vi "Transfer Images Data to UI.vi"(0 "fpga interface in":refnum<k20>, 1 "'stop' notifier":refnum<notifier>, 3 "measure call context in":refnum<class "Measure Call Context.lvclass">, 5 "Active Channel":string[](array[string]), 11 "error in":errorcluster, 12 "References":T1, 13 "raw display notifier":refnum<notifier>) -> (4 "fpga interface out":refnum<k20>, 15 "error out":errorcluster)   [LabVIEW 2025, in "Automotive Vision.lvclass"]
doc: "Handles frame grabbing, and prepare data for sendig it to the UI."
uses:
  Automotive Vision.lvclass
  Automotive Vision.lvclass/Automotive Vision.ctl
  <vilib>/rvi/interface/nirviReadWriteControl/nirviReadWriteControl.xnode
  deps/NI148X/Getting Started/Host/Common/GettingStarted_Common_148X_Host.lvlib
  deps/NI148X/Getting Started/Host/Common/Types/148x_Common_FPGA_Reference.ctl
  NiFpgaLv.dll
  <vilib>/Utility/error.llb/Error Cluster From Error Code.vi
  <vilib>/rvi/interface/Simulation/niFpgaSimulationCallBeginRW.vi
  <vilib>/rvi/errors/niLvFpgaAdjustHostInterfaceError.vi
  <vilib>/Plug-In SDKs/Measurements/Measure Call Context/Measure Call Context.lvclass
  <instrlib>/FlexRIO/CSI-2/v2/Common/Types/LLP Data Type.ctl
  <instrlib>/FlexRIO/CSI-2/v2/Common/NI CSI-2 API Common v2.lvlib
  Automotive-Vision OOB Data Transfer/Automotive-Vision OOB Data Transfer.lvlib
  Measurement Results.ctl
  <vilib>/vision/Image Controls.llb/IMAQ Image.ctl
  deps/NI148X/Getting Started/Host/Common/Types/RAW Interpretation for Display.ctl
  deps/NI148X/Getting Started/Host/Common/Types/Serial Channel Display Parameters.ctl
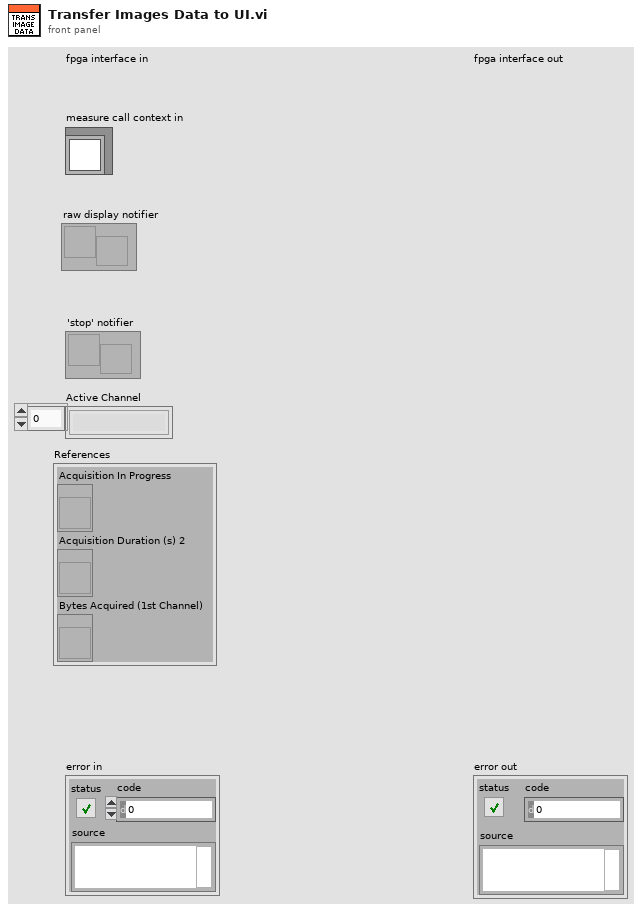
[diagram p1: front panel]
types:
  T1 = cluster{"Acquisition In Progress":refnum<vi>, "Acquisition Duration (s) 2":refnum<vi>, "Bytes Acquired (1st Channel)":refnum<vi>}
  T2 = typedef "NI CSI-2 API Common v2.lvlib/LLP Data Type.ctl" = enum8{"Frame Start", "Frame End", "Line Start", "Line End", "End of Transmission", "Reserved 0", "Reserved 1", "Reserved 2", "Generic Short Packet 1", "Generic Short Packet 2", "Generic Short Packet 3", "Generic Short Packet 4", "Generic Short Packet 5", "Generic Short Packet 6", "Generic Short Packet 7", "Generic Short Packet 8", "Null", "Blanking Data", "Embedded 8-bit non Image Data", "Generic Long Packet 1", "Generic Long Packet 2", "Generic Long Packet 3", "Generic Long Packet 4", "Reserved 3", "YUV420 8-bit", "YUV420 10-bit", "Legacy YUV420 8-bit", "Reserved 4", "YUV420 8-bit Chroma Shifted", "YUV420 10-bit Chroma Shifted", "YUV422 8-bit", "YUV422 10-bit", "RGB444", "RGB555", "RGB565", "RGB666", "RGB888", "Reserved 5", "Reserved 6", "RAW 24", "RAW 6", "RAW 7", "RAW 8", "RAW 10", "RAW 12", "RAW 14", "RAW 16", "RAW 20", "User Defined 8-bit Data 1", "User Defined 8-bit Data 2", "User Defined 8-bit Data 3", "User Defined 8-bit Data 4", "User Defined 8-bit Data 5", "User Defined 8-bit Data 6", "User Defined 8-bit Data 7", "User Defined 8-bit Data 8", "USL Command", "Reserved 7", "Reserved 8", "Reserved 9", "Reserved 10", "Reserved 11", "Reserved 12", "LRTE EPD Spacer"}
  T3 = cluster{"serial channel":fxp<+,3,3>, "frame number":u16, "data type":T2, "width":u16, "height":u16, "image bytes":u32, "total bytes":u32, "little endian":bool, "Status":string}
  T4 = typedef "GettingStarted_Common_148X_Host.lvlib/148x_Common_FPGA_Reference.ctl" = refnum<k20>
  T5 = typedef "GettingStarted_Common_148X_Host.lvlib/Serial Channel Display Parameters.ctl" = cluster{"images":cluster{"grayscale":T6, "color":T6}, "RAW parameters":cluster{"interpretation":T7, "bayer parameters":cluster{"pattern":i32, "algorithm":i32, "red gain":dbl, "green gain":dbl, "blue gain":dbl}}}
  T6 = typedef "IMAQ Image.ctl" = refnum<image>
  T7 = typedef "GettingStarted_Common_148X_Host.lvlib/RAW Interpretation for Display.ctl" = enum16{"Grayscale", "Bayer", "RGB", "YUV422", "YUV420", "Legacy YUV420"}
  T8 = typedef "GettingStarted_Common_148X_FPGA.lvlib/Image Metadata.ctl" = cluster{"serial channel":fxp<+,3,3>, "frame number":u16, "data type":T2, "width":u16, "height":u16, "image bytes":u32, "total bytes":u32, "little endian":bool}
  T9 = typedef "Automotive-Vision OOB Data Transfer.lvlib/OOB to Logic Data.ctl" = cluster{"PauseResume":bool, "ExportPath":string, "ExportType":u16, "Export":bool}
  T10 = typedef "Automotive Vision.lvclass/Measurement Results.ctl" = cluster{"ACQ. IN PROGRESS":bool, "IMAGE PIXEL DATA":u32[], "ACQ. DURATION (s)":dbl, "SOURCE RATE (fps)":dbl, "BYTES ACQUIRED":u64, "FRAME COUNT":u64, "POC VOLTAGE (V)":dbl, "POC CURRENT (A)":dbl, "ERROR":bool, "STATE MESSAGE":string, "IMAGE DATA":string, "OOB gRPC Port":i32, "HEIGHT":u64, "WIDTH":u64}
  T11 = cluster{"image pixel data fifo overflow":bool, "image metadata fifo overflow":bool}[]
  T12 = cluster{"image pixel data fifo overflow":bool, "image metadata fifo overflow":bool}
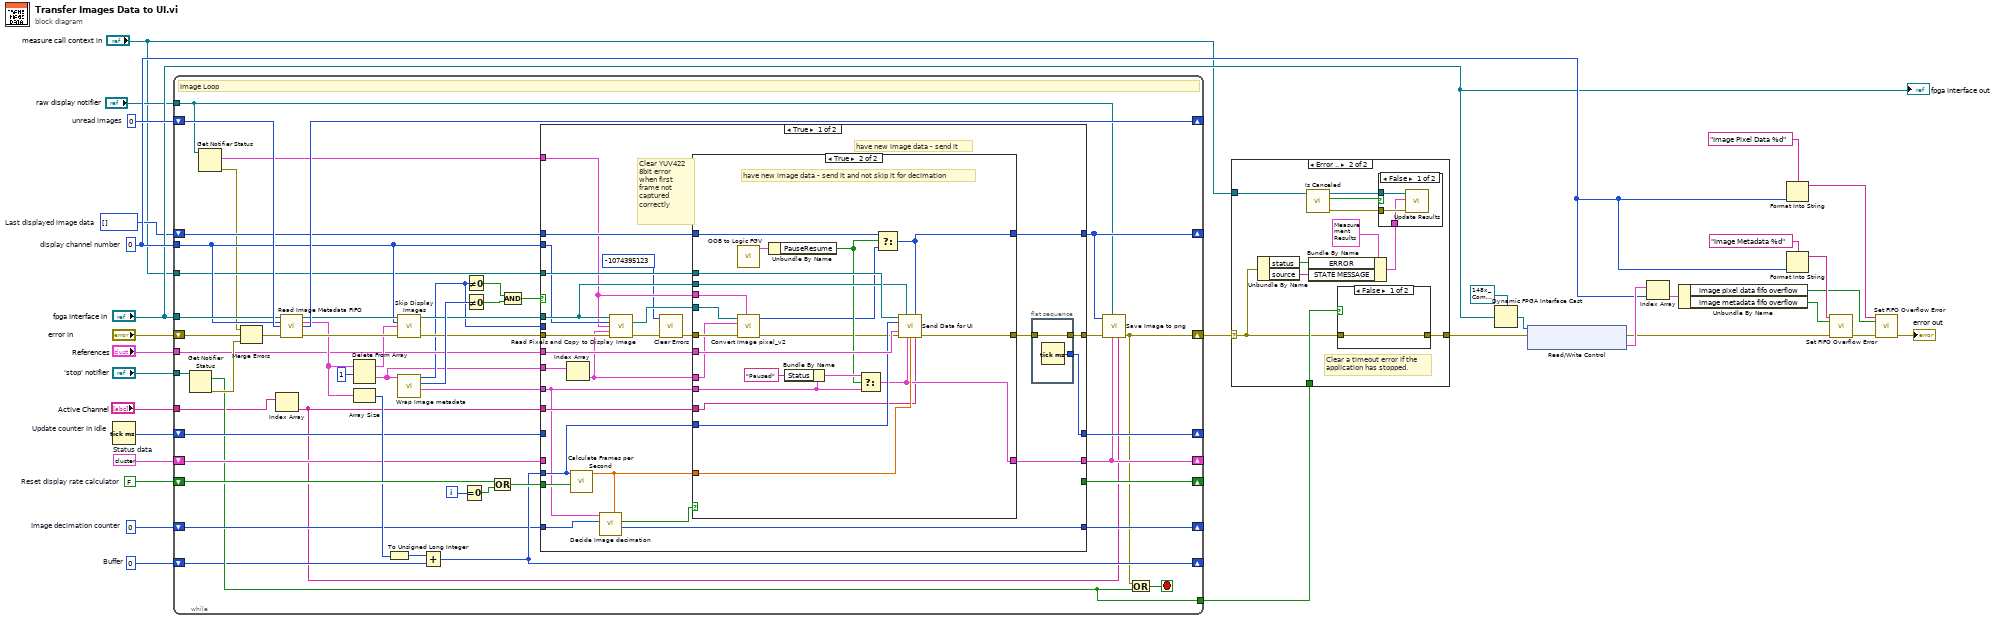
[diagram p0: block diagram]
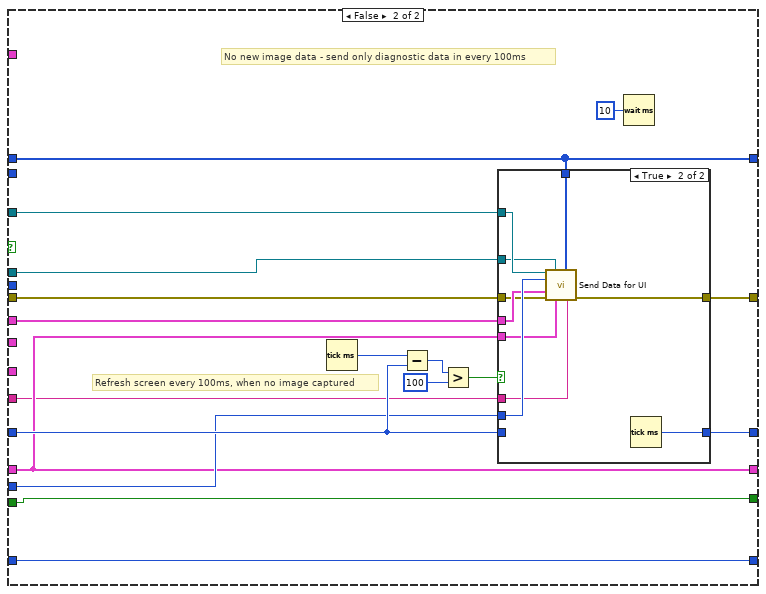
[diagram p3: hidden frame]
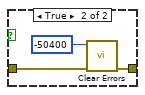
[diagram p7: hidden frame]
diagram:
  w4 = T3 {"serial channel"=0.0, "frame number"=0, "data type"=enum."Frame Start", "width"=0, "height"=0, "image bytes"=0, "total bytes"=0, "little endian"=FALSE, "Status"="Ready for Acquisition"}  # Status data
  w22 = 0  # display channel number
  w7 = u32 0  # Image decimation counter
  w8 = u32[] []  # Last displayed image data
  w14 = u32 0  # Buffer
  w15 = FALSE  # Reset display rate calculator
  w31 = u32 0  # unread images
  n1 = Tick Count (ms) "Update counter in Idle"() -> (millisecond timer value=w9:u32)
  n2 = while {
    shift-right: [w38] -> w13
    shift-left: "error in" -> [w56]
    tunnel: "fpga interface in" -> [w59]
    shift-right: [w79] -> _
    shift-left: w31 -> [w70]
    tunnel: w22 -> [w55]
    shift-right: [w74] -> _
    shift-left: w15 -> [w71]
    shift-right: [w61] -> _
    shift-left: w14 -> [w42]
    tunnel: [w44] -> w11
    tunnel: "'stop' notifier" -> [w58]
    shift-right: [w53] -> _
    shift-left: w9 -> [w54]
    shift-right: [w41] -> _
    shift-left: w8 -> [w52]
    shift-right: [w50] -> _
    shift-left: w7 -> [w51]
    tunnel: "References" -> [w49]
    tunnel: "measure call context in" -> [w48]
    shift-right: [w39] -> _
    shift-left: w4 -> [w47]
    tunnel: "raw display notifier" -> [w35]
    tunnel: "Active Channel" -> [w37]
    i -> [w78]
    stop <- w80 stop-if-true
    # "Image Loop"
    n3 = Get Notifier Status(notifier=w58) -> (current notification=w44:bool, error out=w81:errorcluster)  [unwired: 1 in, 3 out]
    n4 = Get Notifier Status(notifier=w35) -> (current notification=w33:T5[], error out=w34:errorcluster)  [unwired: 1 in, 3 out]
    n5 = Merge Errors(w34, w56, w81) -> (w57:errorcluster)
    n6 = Index Array(array=w37) -> (element=w36:string)  [unwired: 1 in]
    n7 = call "Read Image Metadata FIFO.vi"("fpga inteface in"=w59, "display channel number"=w55, "number of images"=w70, "error in (no error)"=w57) -> ("fpga interface out"=w67:refnum<k20>, "image metadata"=w60:T8[], "images remaining"=w79:u32, "error out"=w64:errorcluster)  [unwired: 8 in]
    n8 = Delete From Array(array=w60, length=1) -> (deleted portion=w32:T8[], array with subset deleted=w63:T8[])  [unwired: 1 in]
    n9 = Array Size(array=w60) -> (size(s)=w62:i32)
    n10 = To Unsigned Long Integer(number=w62) -> (unsigned 32bit integer=w43:u32)
    n11 = call "Skip Display Images.vi"("fpga interface in"=w67, "display channel number"=w55, "image metadata"=w63, "error in (no error)"=w64) -> ("fpga interface out"=w66:refnum<k20>, "error out"=w65:errorcluster)  [unwired: 10 in]
    n12 = call "Wrap Image metadata.vi"("image metadata"=w32) -> ("element"=w46:T3, "Numeric"=w69:i32, "total bytes"=w45:u32)  [unwired: 8 in]
    n13 = Add(x=w43, y=w42) -> (x+y=w61:u32)
    n14 = Equal To 0?(x=w78) -> (x = 0?=w72:bool)
    n15 = Not Equal To 0?(x=w45) -> (x != 0?=w76:bool)
    n16 = Not Equal To 0?(x=w69) -> (x != 0?=w77:bool)
    n17 = Compound Arithmetic op=OR(w71, w72) -> (w73:bool)
    n18 = Compound Arithmetic op=AND(w76, w77) -> (w75:bool)
    n19 = case shown="True" w75 {
      tunnel: w65 -> [w93 w136]
      tunnel: w66 -> [w92 w134]
      tunnel: w55 -> [w91 _]
      tunnel: [w105 w143] -> w40
      tunnel: w73 -> [w96 w150]
      tunnel: [_ w150] -> w74
      tunnel: w61 -> [w102 w140]
      tunnel: w45 -> [_ _]
      tunnel: w46 -> [w86 _]
      tunnel: w48 -> [w107 w137]
      tunnel: w49 -> [w106 w151]
      tunnel: w54 -> [_ w142]
      tunnel: [w104 w144] -> w53
      tunnel: w52 -> [w101 w141]
      tunnel: [w103 w141] -> w41
      tunnel: w51 -> [w100 w139]
      tunnel: [w99 w139] -> w50
      tunnel: w47 -> [_ w138]
      tunnel: [w97 w138] -> w39
      tunnel: w36 -> [w95 w135]
      tunnel: w33 -> [w87 _]
      tunnel: w32 -> [w90 _]
      frame True {
        # "Clear YUV422 8bit error when first frame not captured correctly"
        # "have new image data - send it"
        n20 = Index Array(array=w90) -> (element=w89:T8)  [unwired: 1 in]
        n21 = call <vilib>:"Calculate Frames per Second.vi"("Reset"=w96, "Buffer Number"=w102) -> ("Acquired Frames/s"=w85:dbl)  [unwired: 7 in, 2 out]
        n22 = call "Decide Image decimation.vi"("FPS"=w85, "Image decimation counter in"=w100, "element in"=w86) -> ("Image decimation counter out"=w99:u32, "send current image data"=w98:bool)  [unwired: 7 in]
        n23 = call "Read Pixels and Copy to Display Image.vi"("fpga interface in"=w92, "display channel number"=w91, "serial channel display parameters"=w87, "image metadata"=w89, "error in (no error)"=w93) -> ("display image"=w88:T6, "error out"=w83:errorcluster)  [unwired: 8 in, 1 out]
        n24 = call <vilib>:"Clear Errors.vi"("error in (no error)"=w83, "specific error code to clear (0: all)"=-1074395123) -> ("error out"=w82:errorcluster)  [unwired: 4 in, 1 out]
        n25 = case shown="True" w98 {
          tunnel: [w108 w123] -> w94
          tunnel: w85 -> [_ w131]
          tunnel: w86 -> [w109 w118]
          tunnel: w107 -> [_ w130]
          tunnel: w106 -> [_ w129]
          tunnel: [w110 w128] -> w103
          tunnel: w102 -> [_ w127]
          tunnel: w101 -> [w110 w126]
          tunnel: [w109 w125] -> w97
          tunnel: w92 -> [_ w124]
          tunnel: w95 -> [_ w117]
          tunnel: w82 -> [w108 w116]
          tunnel: w88 -> [_ w114]
          tunnel: w89 -> [_ w112]
          tunnel: w87 -> [_ w111]
          frame False {
            # "have new image data - but skip the sending to not overload UI with data transfer"
          }
          frame True {
            # "have new image data - send it and not skip it for decimation"
            n26 = call "OOB to Logic FGV.vi"() -> ("OOB to Logic Data out"=w120:T9)  [unwired: 10 in, 1 out]
            n27 = call "Convert Image pixel_v2.vi"("serial channel display parameters"=w111, "error in"=w116, "image metadata"=w112, "Refnum in"=w114) -> ("error out"=w115:errorcluster, "Image Pixels (U32)"=w113:u32[])  [unwired: 6 in]
            n28 = Unbundle By Name(w120) -> ("PauseResume"=w119:bool)
            n29 = Bundle By Name(cluster=w118, "Status"="Paused") -> (w122:T3)
            n30 = Select(t=w122, s=w119, f=w118) -> (s? t:f=w125:T3)
            n31 = Select(t=w126, s=w119, f=w113) -> (s? t:f=w128:u32[])
            n32 = call "Send Data for UI.vi"("Measure Call Context in"=w130, "fpga interface in"=w124, "Last displayed image data"=w128, "FrameCount"=w127, "References"=w129, "error in"=w115, "Status data"=w125, "SOURCE RATE (fps)"=w131, "Active Channel"=w117) -> ("error out"=w123:errorcluster)  [unwired: 6 in]
          }
        }
        n33 = flat-sequence {
          tunnel: [w133] -> w105
          tunnel: w94 -> [w133]
          tunnel: [w132] -> w104
          frame #0 {
            n34 = Tick Count (ms)() -> (millisecond timer value=w132:u32)
          }
        }
      }
      frame False {
        # "Refresh screen every 100ms, when no image captured"
        # "No new image data - send only diagnostic data in every 100ms"
        n35 = Tick Count (ms)() -> (millisecond timer value=w148:u32)
        n36 = Subtract(x=w148, y=w142) -> (x-y=w147:u32)
        n37 = Greater?(x=w147, y=u32 100) -> (0:w145:bool)
        n38 = case shown="True" w145 {
          tunnel: w136 -> [w153 w156]
          tunnel: [w153 w163] -> w143
          tunnel: w138 -> [_ w158]
          tunnel: w151 -> [_ w159]
          tunnel: [w152 w162] -> w144
          tunnel: w142 -> [w152 _]
          tunnel: w141 -> [_ w161]
          tunnel: w140 -> [_ w160]
          tunnel: w137 -> [_ w157]
          tunnel: w135 -> [_ w155]
          tunnel: w134 -> [_ w154]
          frame False {
          }
          frame True {
            n39 = call "Send Data for UI.vi"("Measure Call Context in"=w157, "fpga interface in"=w154, "Last displayed image data"=w161, "FrameCount"=w160, "References"=w159, "error in"=w156, "Status data"=w158, "Active Channel"=w155) -> ("error out"=w163:errorcluster)  [unwired: 7 in]
            n40 = Tick Count (ms)() -> (millisecond timer value=w162:u32)
          }
        }
        n41 = Wait (ms)(milliseconds to wait=u32 10) -> ()  [unwired: 1 out]
      }
    }
    n42 = call "Save Image to png.vi"("Channel"=w36, "image metadata"=w39, "raw display notifier"=w35, "error in"=w40, "Last displayed image data"=w41) -> ("error out"=w38:errorcluster)  [unwired: 6 in]
    n43 = Compound Arithmetic op=OR(w38, w44) -> (w80:bool)
  }
  n44 = case shown="Error .." w13 {
    selector: w13 -> [w164 w168]
    tunnel: [w164 w175] -> w26
    tunnel: w11 -> [_ w174]
    tunnel: "measure call context in" -> [_ w165]
    frame No Error {
    }
    frame Error {
      # "Clear a timeout error if the application has stopped."
      n45 = Unbundle By Name(w168) -> ("status"=w167:bool, "source"=w166:string)
      n46 = call <vilib>:"Is Canceled.vi"("measure call context in"=w165) -> ("error out"=w172:errorcluster, "is canceled?"=w171:bool, "measure call context out"=w173:refnum<class "Measure Call Context.lvclass">)  [unwired: 8 in]
      n47 = Bundle By Name(cluster=T10 {"ACQ. IN PROGRESS"=FALSE, "IMAGE PIXEL DATA"=[], "ACQ. DURATION (s)"=0.0, "SOURCE RATE (fps)"=0.0, "BYTES ACQUIRED"=0, "FRAME COUNT"=0, "POC VOLTAGE (V)"=0.0, "POC CURRENT (A)"=0.0, "ERROR"=FALSE, "STATE MESSAGE"="", "IMAGE DATA"="", "OOB gRPC Port"=0, "HEIGHT"=0, "WIDTH"=0} ("Measurement Results"), "ERROR"=w167, "STATE MESSAGE"=w166) -> (w169:T10)
      n48 = case shown="False" w174 {
        tunnel: w168 -> [w179 w182]
        tunnel: [w179 w180] -> w175
        frame False {
        }
        frame True {
          n49 = call <vilib>:"Clear Errors.vi"("error in (no error)"=w182, "specific error code to clear (0: all)"=-50400 ("y")) -> ("error out"=w180:errorcluster)  [unwired: 4 in, 1 out]
        }
      }
      n50 = case shown="False" w171 {
        tunnel: w173 -> [w178 _]
        tunnel: w172 -> [w177 _]
        tunnel: w169 -> [w176 _]
        frame False {
          n51 = call <vilib>:"Update Results.vi"("error in"=w177, "measurement results"=w176, "measure call context in"=w178) -> ()  [unwired: 7 in, 2 out]
        }
        frame True {
        }
      }
    }
  }
  n52 = Dynamic FPGA Interface Cast(Session In=T4 refnum ("FPGA VI Reference Out"), Type="fpga interface in") -> (Session Out=w27:T4)
  n53 = xnode ("Read/Write Control")("FPGA VI Reference In"=w27, "error in"=w26) -> ("error out"=w25:errorcluster, "display channel status"=w29:T11)  [unwired: 1 out]
  n54 = Index Array(array=w29, index=w22) -> (element=w30:T12)
  n55 = Unbundle By Name(w30) -> ("image pixel data fifo overflow"=w17:bool, "image metadata fifo overflow"=w16:bool)
  n56 = Format Into String(format string="Image Pixel Data %d", w22) -> (resulting string=w19:string)  [unwired: 2 in, 1 out]
  n57 = Format Into String(format string="Image Metadata %d", w22) -> (resulting string=w18:string)  [unwired: 2 in, 1 out]
  n58 = call "Set FIFO Overflow Error.vi"("fifo name"=w18, "overflow"=w16, "error in (no error)"=w25) -> ("error out"=w21:errorcluster)  [unwired: 12 in]
  n59 = call "Set FIFO Overflow Error.vi"("fifo name"=w19, "overflow"=w17, "error in (no error)"=w21) -> ("error out"=→"error out":errorcluster)  [unwired: 12 in]
  "fpga interface out" <- "fpga interface in"
